vi "BaseProvider_GetDesignPatternMethods.vi"(1 "DesignPattern":T1[](array[typedef]), 2 "ClassTemplateName":string, 3 "ConnectorPaneSettings":string, 5 "error in":errorcluster) -> (15 "NormalMethods":T3[](array[typedef]), 19 "error out":errorcluster)   [LabVIEW 2020]
uses:
  Provider_LvNativeClass/ClassWriterNative_class/MethodInfo.ctl
  Provider_LvNativeClass/ClassWriterNative_class/MethodType.ctl
  Provider_LvNativeClass/ClassWriterNative_class/MethodInfo_Option.ctl
  Common/LvClass_class/GDSLvClass_PlugIn.ctl
  Common/LvClass_class/GDSLvClass_PlugInTypes.ctl
  <vilib>/Utility/config.llb/Read Key (String).vi
  <vilib>/Utility/config.llb/NI_LVConfig.lvlib
  Provider_LvNativeClass/ClassWriterNative_class/ClassWriterNative.lvclass
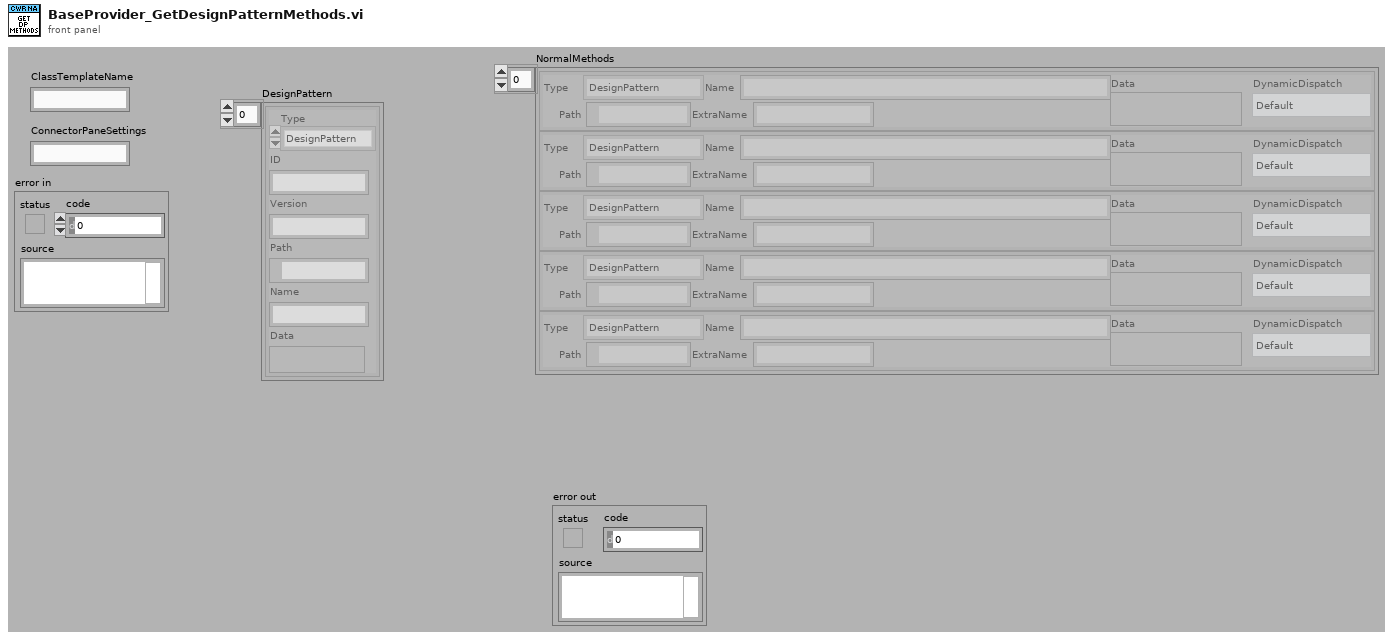
[diagram p1: front panel]
types:
  T1 = typedef "GDSLvClass_PlugIn.ctl" = cluster{"Type":T2, "ID":string, "Version":string, "Path":path, "Name":string, "Data":variant}
  T2 = typedef "GDSLvClass_PlugInTypes.ctl" = enum16{"DesignPattern", "MethodTypes"}
  T3 = typedef "ClassWriterNative.lvclass/MethodInfo.ctl" = cluster{"Type":T4, "Name":string, "Path":path, "ExtraName":string, "Data":variant, "DynamicDispatch":T5}
  T4 = typedef "ClassWriterNative.lvclass/MethodType.ctl" = enum16{"Normal", "MethodPlugIn", "DesignPattern", "AF-Method"}
  T5 = typedef "ClassWriterNative.lvclass/MethodInfo_Option.ctl" = enum16{"Default", "OnAtStart", "OffAtStart", "AlwaysOn", "AlwaysOff"}
  T6 = typedef "NI_LVConfig.lvlib/Config Data RefNum.ctl" = refnum<k1>
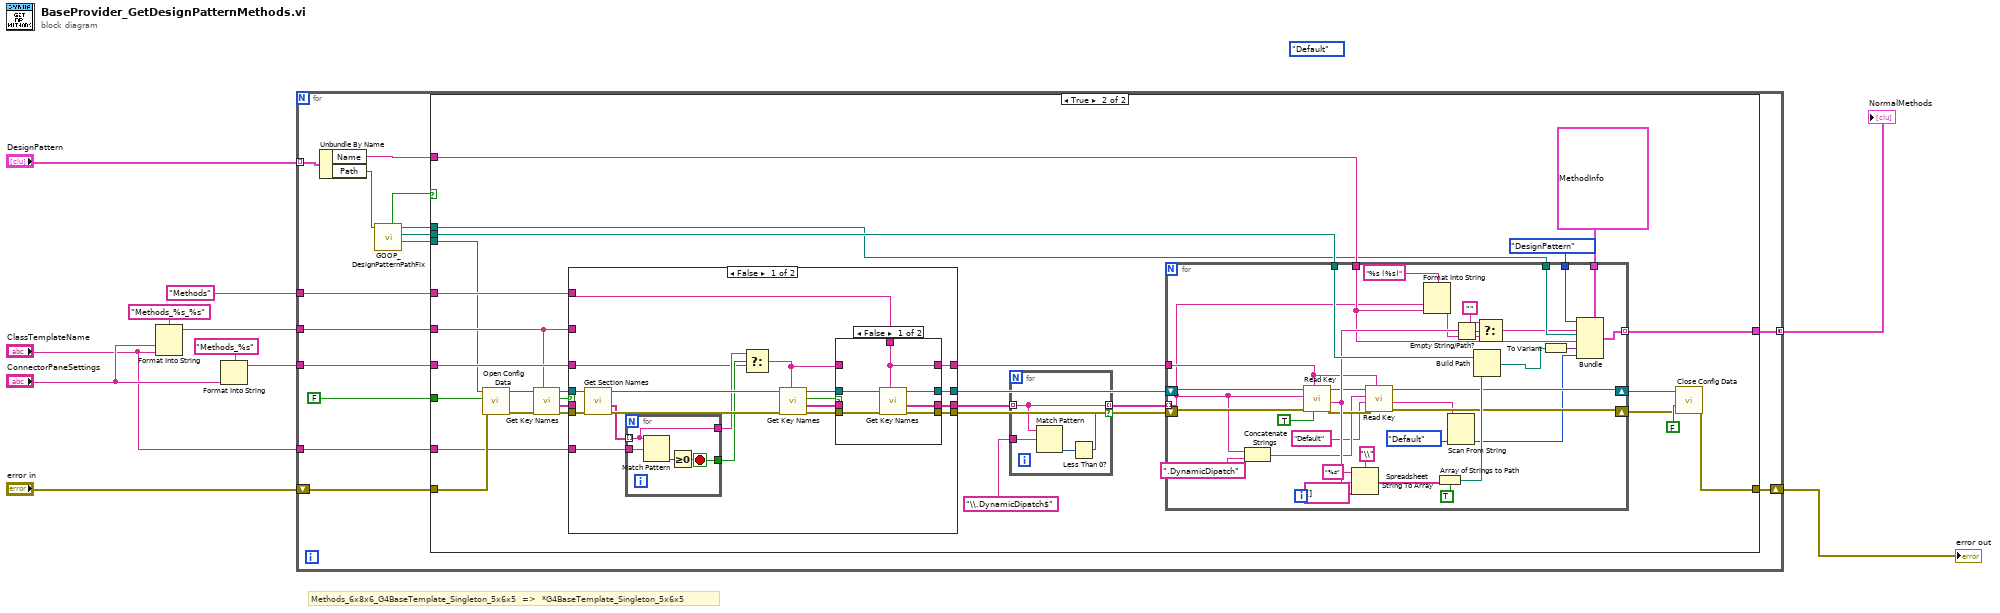
[diagram p0: block diagram]
diagram:
  (unwired) MethodInfo_Option."Default" ("DynamicDispatch")
  # "Methods_6x8x6_G4BaseTemplate_Singleton_5x6x5  =>  *G4BaseTemplate_Singleton_5x6x5"
  n1 = Format Into String(format string="Methods_%s_%s" ("section"), "ConnectorPaneSettings", "ClassTemplateName") -> (resulting string=w4:string)  [unwired: 2 in, 1 out]
  n2 = Format Into String(format string="Methods_%s" ("section"), "ConnectorPaneSettings") -> (resulting string=w7:string)  [unwired: 2 in, 1 out]
  n3 = for {
    shift-right: [w18] -> w10
    shift-left: "error in" -> [w26]
    tunnel: "DesignPattern" -> [w24] mode=indexing
    tunnel: w7 -> [w21]
    tunnel: w4 -> [w19]
    tunnel: "Methods" ("section") -> [w20]
    tunnel: [w13] -> w2 mode=concatenating
    tunnel: "ClassTemplateName" -> [w12]
    n4 = Unbundle By Name(w24) -> ("Name"=w23:string, "Path"=w16:path)
    n5 = call "GOOP_DesignPatternPathFix.vi"("ViPathIn"=w16) -> ("Ini-File"=w17:path, "Folder"=w22:path, "ViPathOut"=w15:path, "Found"=w14:bool)  [unwired: 6 in, 1 out]
    n6 = case shown="True" w14 {
      tunnel: w26 -> [w27 w56]
      tunnel: FALSE ("create file if necessary? (T)") -> [_ w54]
      tunnel: w23 -> [_ w47]
      tunnel: w22 -> [_ w46]
      tunnel: w21 -> [_ w44]
      tunnel: w20 -> [_ w37]
      tunnel: w19 -> [_ w36]
      tunnel: [w27 w35] -> w18
      tunnel: w17 -> [_ w34]
      tunnel: w15 -> [_ w33]
      tunnel: [_ w32] -> w13
      tunnel: w12 -> [_ w28]
      frame False {
      }
      frame True {
        n7 = call <vilib>:"Open Config Data.vi"("error in (no error)"=w56, "create file if necessary (T)"=w54, "configuration file path"=w34) -> ("error out"=w43:errorcluster, "refnum"=w42:T6)  [unwired: 6 in, 1 out]
        n8 = call <vilib>:"Get Key Names.vi"("section"=w36, "error in (no error)"=w43, "refnum"=w42) -> ("error out"=w41:errorcluster, "key names"=w38:string[], "section exists?"=w39:bool, "refnum out"=w40:T6)  [unwired: 5 in]
        n9 = case shown="False" w39 {
          tunnel: [w79 w97] -> w31
          tunnel: [w78 w96] -> w53
          tunnel: [w77 w95] -> w52
          tunnel: [w72 w94] -> w45
          tunnel: w44 -> [w62 _]
          tunnel: w41 -> [w70 w95]
          tunnel: w40 -> [w69 w96]
          tunnel: w38 -> [_ w97]
          tunnel: w37 -> [w71 _]
          tunnel: w36 -> [_ w94]
          tunnel: w28 -> [w65 _]
          frame False {
            n10 = call <vilib>:"Get Section Names.vi"("error in (no error)"=w70, "refnum"=w69) -> ("error out"=w67:errorcluster, "section names"=w66:string[], "refnum out"=w68:T6)  [unwired: 7 in]
            n11 = for {
              tunnel: w66 -> [w80] mode=indexing
              tunnel: w65 -> [w83]
              tunnel: [w81] -> w64
              tunnel: [w80] -> w63
              stop <- w81 stop-if-true
              n12 = Match Pattern(string=w80, regular expression=w83) -> (offset past match=w82:i32)  [unwired: 1 in, 3 out]
              n13 = Greater Or Equal To 0?(x=w82) -> (x >= 0?=w81:bool)
            }
            n14 = Select(t=w63, s=w64, f=w62) -> (s? t:f=w61:string)
            n15 = call <vilib>:"Get Key Names.vi"("section"=w61, "error in (no error)"=w67, "refnum"=w68) -> ("error out"=w74:errorcluster, "key names"=w73:string[], "section exists?"=w75:bool, "refnum out"=w76:T6)  [unwired: 5 in]
            n16 = case shown="False" w75 {
              tunnel: [w89 w93] -> w79
              tunnel: [w88 w92] -> w78
              tunnel: [w87 w91] -> w77
              tunnel: w76 -> [w86 w92]
              tunnel: w74 -> [w85 w91]
              tunnel: w73 -> [_ w93]
              tunnel: [w84 w90] -> w72
              tunnel: w61 -> [_ w90]
              tunnel: w71 -> [w84 _]
              frame False {
                n17 = call <vilib>:"Get Key Names.vi"("section"=w84, "error in (no error)"=w85, "refnum"=w86) -> ("error out"=w87:errorcluster, "key names"=w89:string[], "refnum out"=w88:T6)  [unwired: 5 in, 1 out]
              }
              frame True {
              }
            }
          }
          frame True {
          }
        }
        n18 = for {
          tunnel: w31 -> [w58] mode=indexing
          tunnel: "\\.DynamicDipatch$" ("string") -> [w60]
          tunnel: [w58] -> w29 mode=indexing if=w57
          n19 = Match Pattern(string=w58, regular expression=w60) -> (offset past match=w59:i32)  [unwired: 1 in, 3 out]
          n20 = Less Than 0?(x=w59) -> (x < 0?=w57:bool)
        }
        n21 = for {
          shift-right: [w106] -> w50
          shift-left: w52 -> [w131]
          shift-right: [w107] -> w51
          shift-left: w53 -> [w132]
          tunnel: w45 -> [w105]
          tunnel: w29 -> [w104] mode=indexing
          tunnel: [w124] -> w32 mode=indexing
          tunnel: w46 -> [w128]
          tunnel: T3 {"Type"=enum."DesignPattern", "Name"="", "Path"=path "", "ExtraName"="", "Data"=variant, "DynamicDispatch"=enum."Default"} ("Cluster") -> [w127]
          tunnel: MethodType."DesignPattern" ("Type") -> [w126]
          tunnel: w33 -> [w125]
          tunnel: w47 -> [w112]
          n22 = Concatenate Strings(w104, ".DynamicDipatch" ("string")) -> (w102:string)
          n23 = call-poly <vilib>:"Read Key.vi"("read raw string? (F)"=TRUE, "section"=w105, "error in (no error)"=w131, "key"=w104, "refnum"=w132) -> ("error out"=w108:errorcluster, "value"=w115:string, "refnum out"=w109:T6)  [unwired: 3 in, 1 out]
          n24 = Spreadsheet String To Array(delimiter (Tab)="\\", format string="%s", spreadsheet string=w115, array type (2D Dbl)=string[] []) -> (array=w116:string[])
          n25 = call-poly <vilib>:"Read Key.vi"("section"=w105, "error in (no error)"=w108, "default value"="Default", "key"=w102, "refnum"=w109) -> ("error out"=w106:errorcluster, "value"=w100:string, "refnum out"=w107:T6)  [unwired: 3 in, 1 out]
          n26 = Format Into String(format string="%s (%s)", w104, w112) -> (resulting string=w110:string)  [unwired: 2 in, 1 out]
          n27 = Array of Strings to Path(0:w116, 1:TRUE ("relative")) -> (2:w114:path)
          n28 = Scan From String(input string=w100, default 1=MethodInfo_Option."Default" ("DynamicDispatch")) -> (output 1=w98:T5)  [unwired: 3 in, 3 out]
          n29 = Empty String/Path?(string/path=w115) -> (empty?=w130:bool)
          n30 = Build Path(base path=w128, name or relative path=w114) -> (appended path=w123:path)
          n31 = Select(t="", s=w130, f=w110) -> (s? t:f=w122:string)
          n32 = To Variant(anything=w123) -> (Variant=w113:variant)
          n33 = Bundle(cluster=w127, "Type"=w126, "Name"=w122, "Path"=w125, "ExtraName"=w112, "Data"=w113, "DynamicDispatch"=w98) -> (w124:T3)
        }
        n34 = call <vilib>:"Close Config Data.vi"("error in (no error)"=w50, "write file if changed (T)"=FALSE ("create file if necessary? (T)"), "refnum"=w51) -> ("error out"=w35:errorcluster)  [unwired: 7 in, 1 out]
      }
    }
  }
  "NormalMethods" <- w2
  "error out" <- w10
